vi "Use Current Time If Empty.vi"(3 "Time(Empty to Use Current Time)":timestamp) -> (1 "Time out":timestamp)   [LabVIEW 2017]
doc: "Input a timestamp and output it directly when the timestamp is normal, and output the correct timestamp according to the current time when the timestamp is empty."
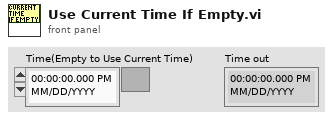
[diagram p1: front panel]
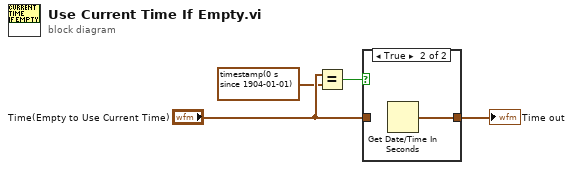
[diagram p0: block diagram]
diagram:
  n1 = Equal?(x="Time(Empty to Use Current Time)", y=timestamp(0 s since 1904-01-01) ("seconds since 1Jan1904")) -> (x = y?=w2:bool)
  n2 = case shown="True" w2 {
    tunnel: [w5 w6] -> w4
    tunnel: "Time(Empty to Use Current Time)" -> [w5 _]
    frame False {
    }
    frame True {
      n3 = Get Date/Time In Seconds() -> (seconds since 1Jan1904=w6:timestamp)
    }
  }
  "Time out" <- w4
